vi "Actor Core.vi"(8 "error in":errorcluster, 11 "ImageHandler:DT-ImageHandler in":refnum<class "DT-ImageHandler.lvclass">) -> (0 "error out":errorcluster, 3 "ImageHandler:DT-ImageHandler out":refnum<class "Actor.lvclass">)   [LabVIEW 2022 SP3, in "ImageHandler.lvlib" / "DT-ImageHandler.lvclass"]
doc: "(<B>Filename</B>: Actor Framework.lvlib:Actor.lvclass:Actor Core.vi)\n\nReceives messages to the actor, reacts to them, and initiates any error handling that may shut the actor down.\n\nDescendant classes may override this VI to append parallel tasks for the actor to complete while it handles messages. Overrides use the Call Parent Class Method node."
uses:
  DT-ImageHandler.lvclass
  C:/Program Files/National Instruments/LabVIEW 2025/vi.lib/ActorFramework/Actor/Actor.lvclass
  <vilib>/ActorFramework/Actor/Actor.lvclass
  DT-ImageHandler.lvclass/DT-ImageHandler.ctl
  <vilib>/ActorFramework/Actor/Actor.lvclass/Actor.ctl
  <vilib>/ActorFramework/Message Enqueuer/Message Enqueuer.lvclass/Message Enqueuer.ctl
  ImageHandler - Controller -- Interface/ImageHandler - Controller -- Interface Messages/Log Message Msg/Log Message Msg.lvclass/Log Message Msg.ctl
  ImageHandler Messages/Write Image Msg/Write Image Msg.lvclass/Write Image Msg.ctl
  ImageHandler - Controller -- Interface/ImageHandler - Controller -- Interface Messages/Log Message Msg/Log Message Msg.lvclass
  C:/Program Files/National Instruments/LabVIEW 2025/vi.lib/ActorFramework/Message/Message.lvclass
  ImageHandler Messages/Write Image Msg/Write Image Msg.lvclass
  <vilib>/ActorFramework/Message Enqueuer/Message Enqueuer.lvclass
  BonTechDetector/BonTechDetector.lvlib
  <vilib>/vision/Image Controls.llb/IMAQ Image.ctl
  xPanelWrapperLvLib/xPanelWrapper.lvlib
panel:
  out "time ms":u32
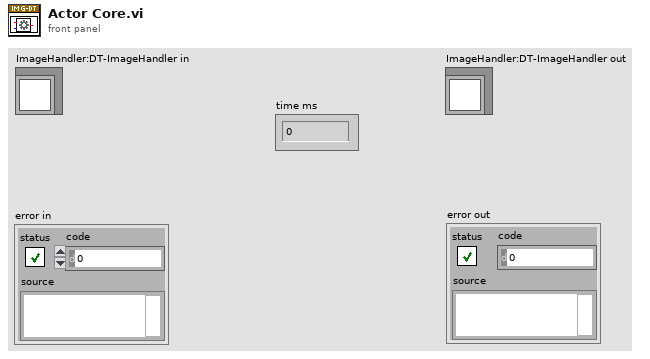
[diagram p1: front panel]
types:
  T1 = cluster{"Init":refnum<user-event>, "DeInit":refnum<user-event>, "Save":refnum<user-event>, "Stop":refnum<user-event>, "Display Mode":refnum<user-event>}
  T2 = cluster{"ImageWriteBuffer":u16[], "Image Width":i32, "Image Height":i32}
  T3 = typedef "IMAQ Image.ctl" = refnum<image>
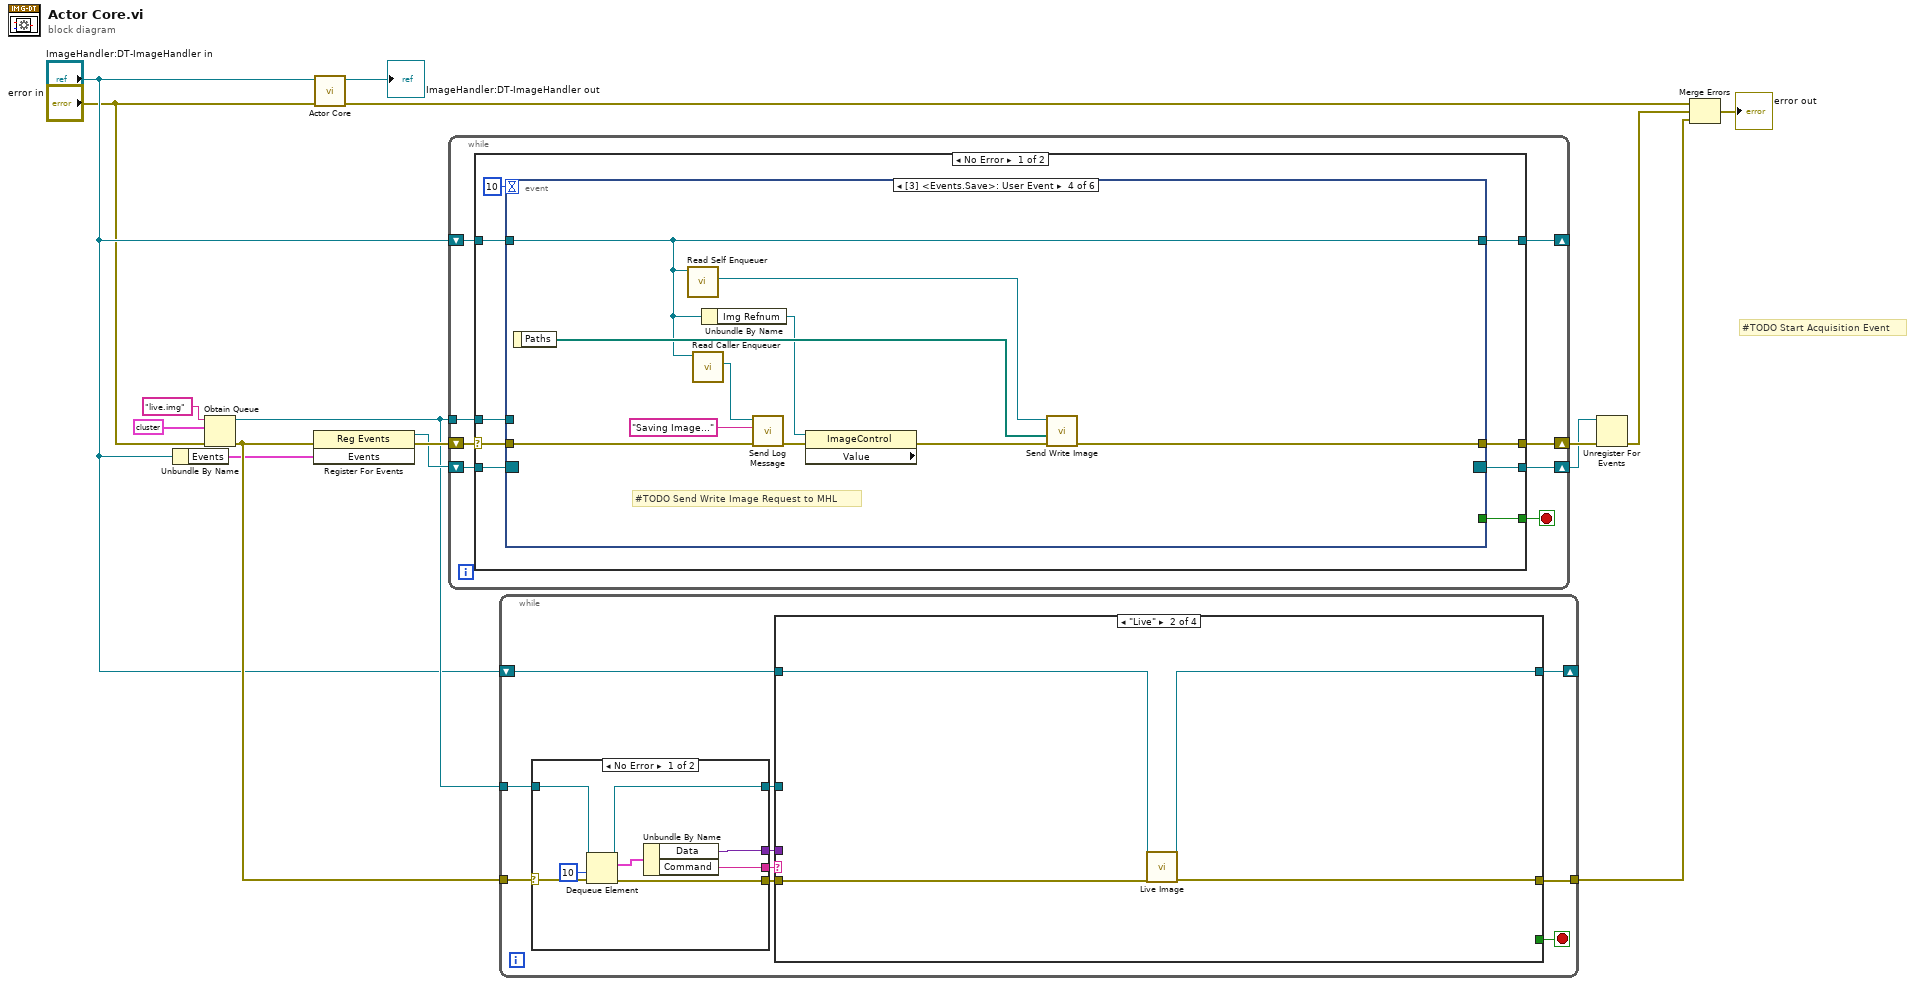
[diagram p0: block diagram]
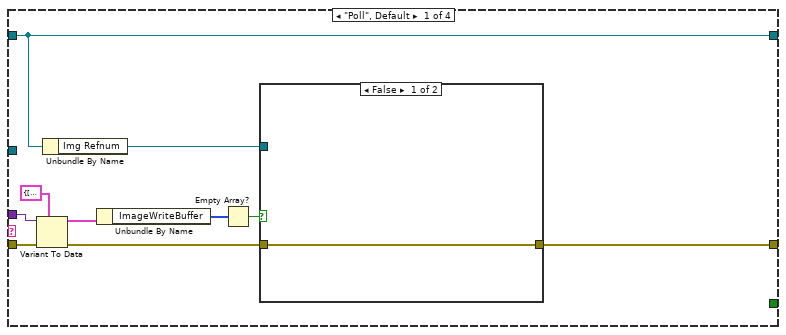
[diagram p2: hidden frame]
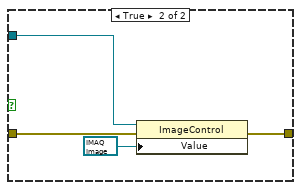
[diagram p3: hidden frame]
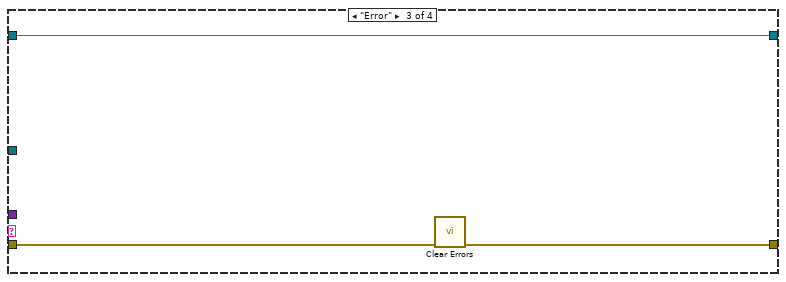
[diagram p4: hidden frame]
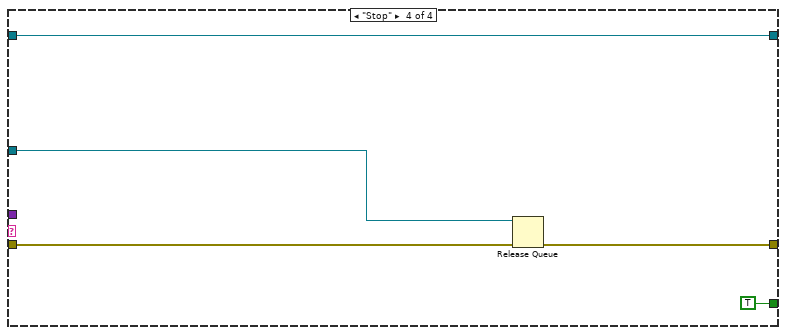
[diagram p5: hidden frame]
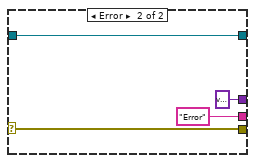
[diagram p6: hidden frame]
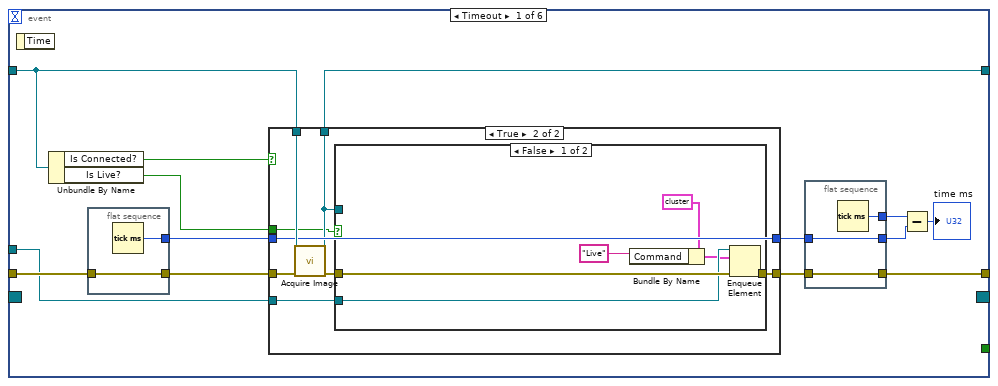
[diagram p7: hidden frame]
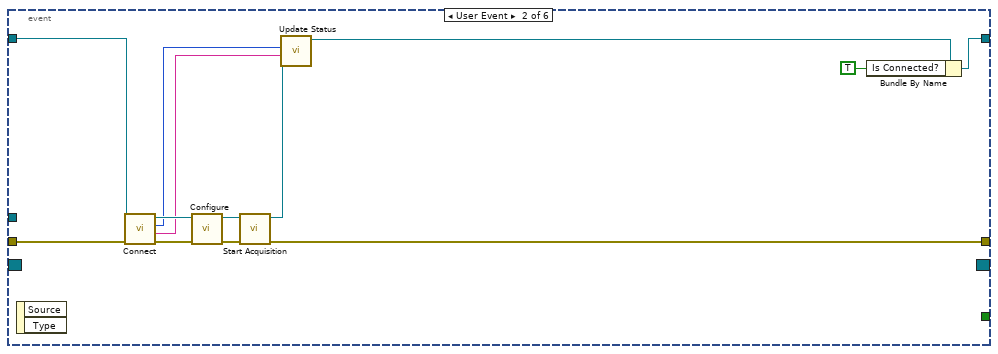
[diagram p10: hidden frame]
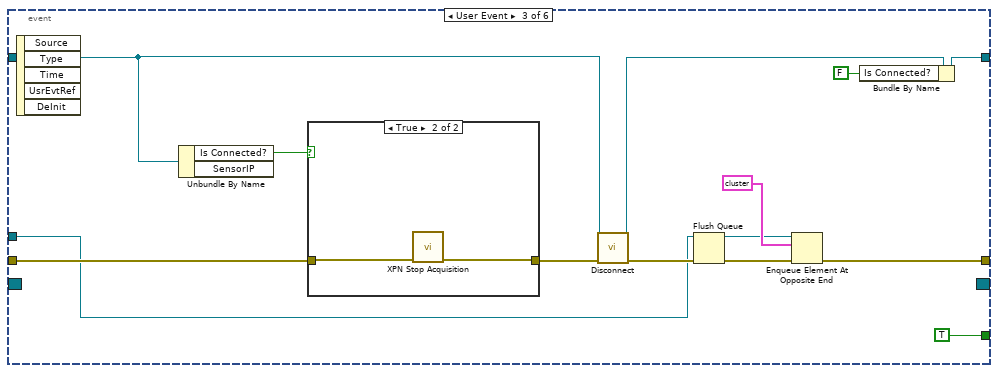
[diagram p11: hidden frame]
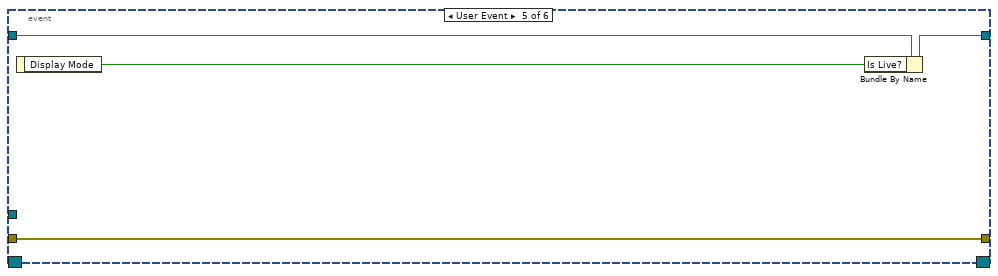
[diagram p13: hidden frame]
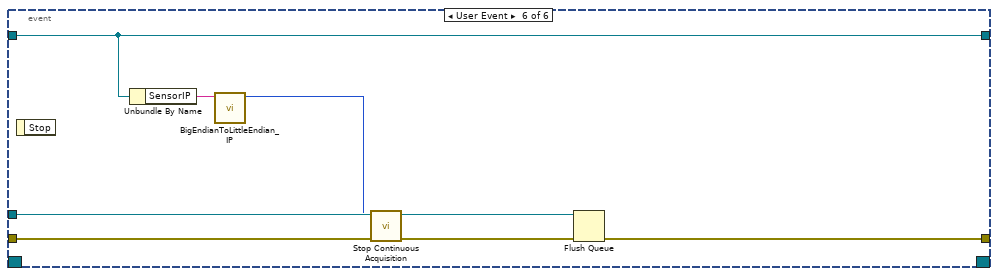
[diagram p14: hidden frame]
diagram:
  # "#TODO Start Acquisition Event"
  n1 = Unbundle By Name("ImageHandler:DT-ImageHandler in") -> ("Events"=w3:T1)
  n2 = Obtain Queue(name (unnamed)="live.img", element data type=cluster{"Data":variant, "Command":string} {"Data"=variant, "Command"=""}, error in (no error)="error in") -> (queue out=w6:refnum<queue>, error out=w5:errorcluster)  [unwired: 2 in, 1 out]
  n3 = register-events(error in=w5, w3) -> (reference out=w13:refnum<event-registration>, error out=w14:errorcluster)  [unwired: 1 in]
  n4 = call-parent "Actor Core.vi"("error in"="error in", "Actor in"="ImageHandler:DT-ImageHandler in") -> ("error out"=w16:errorcluster, "Actor out"=→"ImageHandler:DT-ImageHandler out":refnum<class "Actor.lvclass">)  [unwired: 8 in]
  n5 = while {
    shift-right: [w23] -> _
    shift-left: "ImageHandler:DT-ImageHandler in" -> [w24]
    shift-right: [w22] -> w12
    shift-left: w14 -> [w19]
    shift-right: [w20] -> w11
    shift-left: w13 -> [w21]
    tunnel: w6 -> [w17]
    stop <- w18 stop-if-true
    n6 = case shown="No Error" w19 {
      selector: w19 -> [w27 w122]
      tunnel: w24 -> [w33 w123]
      tunnel: [w32 w123] -> w23
      tunnel: [w31 w122] -> w22
      tunnel: w21 -> [w30 w124]
      tunnel: [w28 w124] -> w20
      tunnel: [w25 _] -> w18
      tunnel: w17 -> [w26 _]
      frame No Error {
        n7 = event shown="[3] <Events.Save>: User Event" {
          selector: w30 -> [_ _ _ _ _ _]
          dyn-events: [_ _ _ _ _ _] -> w28
          timeout: 10 -> [_ _ _ _ _ _]
          tunnel: w27 -> [w44 w83 w96 w105 w111 w120]
          tunnel: w33 -> [w46 w82 w87 w108 w114 w119]
          tunnel: [w47 w72 w94 w108 w113 w119] -> w32
          tunnel: [w40 w78 w89 w101 w111 w117] -> w31
          tunnel: w26 -> [w35 _ w85 _ _ w121]
          tunnel: [_ _ TRUE _ _ _] -> w25
          event Timeout {
            n8 = event-data() -> ()  [unwired: 1 in, 1 out]
            n9 = Unbundle By Name(w46) -> ("Is Connected?"=w45:bool, "Is Live?"=w34:bool)
            n10 = flat-sequence {
              tunnel: w44 -> [w69]
              tunnel: [w70] -> w43
              tunnel: [w69] -> w42
              frame #0 {
                n11 = Tick Count (ms)() -> (millisecond timer value=w70:u32)
              }
            }
            n12 = case shown="True" w45 {
              tunnel: w42 -> [w49 w58]
              tunnel: [w49 w54] -> w41
              tunnel: w46 -> [w50 w56]
              tunnel: [w50 w52] -> w47
              tunnel: w43 -> [w48 w55]
              tunnel: [w48 w55] -> w39
              tunnel: w35 -> [_ w53]
              tunnel: w34 -> [_ w51]
              frame False {
              }
              frame True {
                n13 = call "Acquire Image.vi"("error in (no error)"=w58, "ImageHandler:DT-ImageHandler in"=w56) -> ("error out"=w57:errorcluster, "ImageHandler:DT-ImageHandler out"=w52:refnum<class "DT-ImageHandler.lvclass">)  [unwired: 8 in]
                n14 = case shown="False" w51 {
                  tunnel: w57 -> [w64 w65]
                  tunnel: [w63 w65] -> w54
                  tunnel: w53 -> [w62 _]
                  tunnel: w52 -> [_ _]
                  frame False {
                    n15 = Bundle By Name(cluster=cluster{"Data":variant, "Command":string} {"Data"=variant, "Command"=""} ("element"), "Command"="Live") -> (w61:cluster{"Data":variant, "Command":string})
                    n16 = Enqueue Element(queue=w62, element=w61, error in (no error)=w64) -> (error out=w63:errorcluster)  [unwired: 1 in, 2 out]
                  }
                  frame True {
                  }
                }
              }
            }
            n17 = flat-sequence {
              tunnel: [w68] -> w38
              tunnel: w41 -> [w67]
              tunnel: [w67] -> w40
              tunnel: w39 -> [w66]
              tunnel: [w66] -> w37
              frame #0 {
                n18 = Tick Count (ms)() -> (millisecond timer value=w68:u32)
              }
            }
            n19 = Subtract(x=w38, y=w37) -> (x-y=→"time ms":u32)
          }
          event User Event {
            n20 = event-data() -> ()  [unwired: 1 in, 2 out]
            n21 = call "Connect.vi"("error in (no error)"=w83, "ImageHandler:DT-ImageHandler in"=w82) -> ("error out"=w80:errorcluster, "Serial Number"=w73:string, "Sensor Status"=w74:i32, "ImageHandler:DT-ImageHandler out"=w81:refnum<class "DT-ImageHandler.lvclass">)  [unwired: 6 in]
            n22 = call "Configure.vi"("error in (no error)"=w80, "ImageHandler:DT-ImageHandler in"=w81) -> ("error out"=w79:errorcluster, "ImageHandler:DT-ImageHandler out"=w77:refnum<class "DT-ImageHandler.lvclass">)  [unwired: 8 in]
            n23 = call "Start Acquisition.vi"("error in (no error)"=w79, "ImageHandler:DT-ImageHandler in"=w77) -> ("error out"=w78:errorcluster, "ImageHandler:DT-ImageHandler out"=w76:refnum<class "DT-ImageHandler.lvclass">)  [unwired: 8 in]
            n24 = call "Update Status.vi"("Serial Number"=w73, "Sensor Status"=w74, "ImageHandler:DT-ImageHandler in"=w76) -> ("ImageHandler:DT-ImageHandler out"=w75:refnum<class "DT-ImageHandler.lvclass">)  [unwired: 7 in, 1 out]
            n25 = Bundle By Name(cluster=w75, "Is Connected?"=TRUE) -> (w72:refnum<class "DT-ImageHandler.lvclass">)
          }
          event User Event {
            n26 = event-data() -> ()  [unwired: 1 in, 5 out]
            n27 = Unbundle By Name(w87) -> ("Is Connected?"=w92:bool)  [unwired: 1 out]
            n28 = case shown="True" w92 {
              tunnel: w96 -> [w98 w100]
              tunnel: [w98 w99] -> w95
              frame False {
              }
              frame True {
                n29 = call "XPN Stop Acquisition.vi"("error in (no error)"=w100) -> ("error out"=w99:errorcluster)  [unwired: 9 in, 1 out]
              }
            }
            n30 = call "Disconnect.vi"("error in (no error)"=w95, "ImageHandler:DT-ImageHandler in"=w87) -> ("error out"=w90:errorcluster, "ImageHandler:DT-ImageHandler out"=w97:refnum<class "DT-ImageHandler.lvclass">)  [unwired: 8 in]
            n31 = Flush Queue(queue=w85, error in (no error)=w90) -> (queue out=w84:refnum<queue>, error out=w86:errorcluster)  [unwired: 1 out]
            n32 = Enqueue Element At Opposite End(queue=w84, element=cluster{"Data":variant, "Command":string} {"Data"=variant, "Command"="Stop"}, error in (no error)=w86) -> (error out=w89:errorcluster)  [unwired: 1 in, 2 out]
            n33 = Bundle By Name(cluster=w97, "Is Connected?"=FALSE) -> (w94:refnum<class "DT-ImageHandler.lvclass">)
          }
          event User Event {
            # "#TODO Send Write Image Request to MHL"
            n34 = event-data() -> ("Paths"=w110:path[])  [unwired: 1 in]
            n35 = call <vilib>:"Read Self Enqueuer.vi"("Actor"=w108) -> ("Self Enqueuer"=w109:refnum<class "Message Enqueuer.lvclass">)  [unwired: 10 in]
            n36 = call <vilib>:"Read Caller Enqueuer.vi"("Actor"=w108) -> ("Caller Enqueuer"=w107:refnum<class "Message Enqueuer.lvclass">)  [unwired: 10 in]
            n37 = Unbundle By Name(w108) -> ("Img Refnum"=w102:refnum<vi>)
            n38 = call "Send Log Message.vi"("error in (no error)"=w105, "Log Message"="Saving Image...", "Message Enqueuer"=w107) -> ("error out"=w104:errorcluster)  [unwired: 7 in, 1 out]
            n39 = property class="ImageControl" props=["Value"](reference=w102, error in=w104) -> (error out=w103:errorcluster)  [unwired: 2 out]
            n40 = call "Send Write Image.vi"("error in (no error)"=w103, "Paths"=w110, "Message Enqueuer"=w109) -> ("error out"=w101:errorcluster)  [unwired: 7 in, 1 out]
          }
          event User Event {
            n41 = event-data() -> ("Display Mode"=w112:bool)  [unwired: 1 in]
            n42 = Bundle By Name(cluster=w114, "Is Live?"=w112) -> (w113:refnum<class "DT-ImageHandler.lvclass">)
          }
          event User Event {
            n43 = event-data() -> ()  [unwired: 1 in, 1 out]
            n44 = Unbundle By Name(w119) -> ("SensorIP"=w116:string)
            n45 = call "BigEndianToLittleEndian_IP.vi"("IP String"=w116) -> ("IP Network Order"=w115:u32)  [unwired: 10 in]
            n46 = call "Stop Continuous Acquisition.vi"("error in (no error)"=w120, "nSensorIP"=w115) -> ("error out"=w118:errorcluster)  [unwired: 8 in, 1 out]
            n47 = Flush Queue(queue=w121, error in (no error)=w118) -> (error out=w117:errorcluster)  [unwired: 2 out]
          }
        }
      }
      frame Error {
      }
    }
  }
  n48 = while {
    tunnel: w6 -> [w134]
    shift-right: [w126] -> _
    shift-left: "ImageHandler:DT-ImageHandler in" -> [w127]
    tunnel: w5 -> [w133]
    tunnel: [w129] -> w4
    stop <- w125 stop-if-true
    n49 = case shown="No Error" w133 {
      selector: w133 -> [w169 w171]
      tunnel: w134 -> [w167 w170]
      tunnel: [w163 "Error" ("Command")] -> w132
      tunnel: [w164 variant ("Data")] -> w131
      tunnel: [w168 w171] -> w130
      tunnel: [w166 w170] -> w128
      frame No Error {
        n50 = Dequeue Element(queue=w167, timeout in ms (-1)=10, error in (no error)=w169) -> (queue out=w166:refnum<queue>, element=w165:cluster{"Data":variant, "Command":string}, error out=w168:errorcluster)  [unwired: 1 out]
        n51 = Unbundle By Name(w165) -> ("Data"=w164:variant, "Command"=w163:string)
      }
      frame Error {
      }
    }
    n52 = case shown="\"Live\"" w132 {
      tunnel: w131 -> [w139 _ _ _]
      tunnel: w130 -> [w144 w153 w154 w157]
      tunnel: [w143 w150 w155 w159] -> w129
      tunnel: w128 -> [_ _ _ w158]
      tunnel: w127 -> [w142 w152 w156 w161]
      tunnel: [w142 w151 w156 w161] -> w126
      tunnel: [_ _ _ TRUE] -> w125
      frame "Poll", Default {
        n53 = Variant To Data(error in=w144, type=T2 {"ImageWriteBuffer"=[], "Image Width"=0, "Image Height"=0}, Variant=w139) -> (data=w137:T2, error out=w140:errorcluster)
        n54 = Unbundle By Name(w142) -> ("Img Refnum"=w141:refnum<vi>)
        n55 = Unbundle By Name(w137) -> ("ImageWriteBuffer"=w136:u16[])
        n56 = Empty Array?(array=w136) -> (empty?=w135:bool)
        n57 = case shown="False" w135 {
          tunnel: w140 -> [w145 w149]
          tunnel: [w145 w148] -> w143
          tunnel: w141 -> [_ w147]
          frame False {
          }
          frame True {
            n58 = property class="ImageControl"(reference=w147, error in=w149, "Value"=T3 refnum ("ImaqLiveBuffer")) -> (error out=w148:errorcluster)  [unwired: 1 out]
          }
        }
      }
      frame "Live" {
        n59 = call "Live Image.vi"("error in (no error)"=w153, "ImageHandler:DT-ImageHandler in"=w152) -> ("error out"=w150:errorcluster, "ImageHandler:DT-ImageHandler out"=w151:refnum<class "DT-ImageHandler.lvclass">)  [unwired: 8 in]
      }
      frame "Error" {
        n60 = call <vilib>:"Clear Errors.vi"("error in (no error)"=w154) -> ("error out"=w155:errorcluster)  [unwired: 5 in, 1 out]
      }
      frame "Stop" {
        n61 = Release Queue(queue=w158, error in (no error)=w157) -> (error out=w159:errorcluster)  [unwired: 1 in, 2 out]
      }
    }
  }
  n62 = Unregister For Events(event registration refnum=w11, error in=w12) -> (error out=w7:errorcluster)
  n63 = Merge Errors(w16, w7, w4) -> (→"error out":errorcluster)
